vi "W_connect-string.vi"(8 "error in (no error)":errorcluster caption="错误输入（无错误）", 10 "connect-string":string, 11 "Database_access输入":refnum<class "Database_access.lvclass">) -> (0 "error out":errorcluster caption="错误输出", 3 "Database_access输出":refnum<class "Database_access.lvclass">)   [LabVIEW 2025, in "Database_access.lvclass"]
uses:
  Database_access.lvclass
  Database_access.lvclass/Database_access.ctl
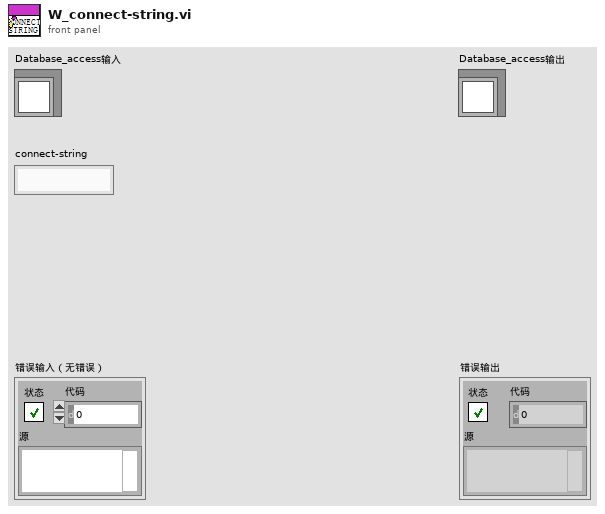
[diagram p1: front panel]
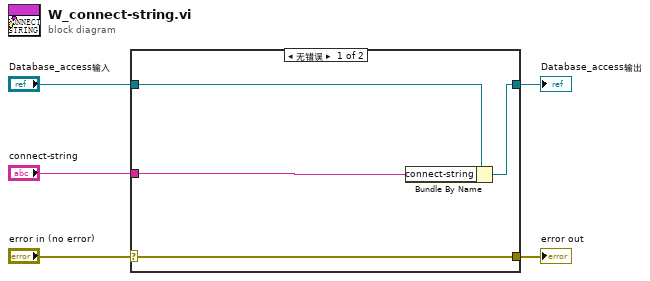
[diagram p0: block diagram]
diagram:
  n1 = case shown="无错误" "error in (no error)" {
    selector: "error in (no error)" -> [w9 w10]
    tunnel: [w9 w10] -> w4
    tunnel: [w7 w11] -> w2
    tunnel: "Database_access输入" -> [w8 w11]
    tunnel: "connect-string" -> [w6 _]
    frame No Error {
      n2 = Bundle By Name(cluster=w8, "connect-string"=w6) -> (w7:refnum<class "Database_access.lvclass">)
    }
    frame Error {
    }
  }
  "error out" <- w4
  "Database_access输出" <- w2
